vi "StateSpaceUtil_MakeCostMatrix.vi"(7 "Elements":i32, 11 "Costs":T1) -> (0 "Sze Coerced":bool, 3 "Costs Matrix":T1)   [LabVIEW 2019, in "Trajectory_Library.lvlib"]
doc: "Creates a cost matrix from the given vector for use with LQR.\n\nThe cost matrix is constructed using Bryson's rule. The inverse square of each tolerance is placed on the cost matrix diagonal. If a tolerance is infinity, its cost matrix entry is set to zero.\n \nInputs:\n - Elements -- representing the number of system states or inputs\n - tolerances -- For a Q matrix, its elements are the maximum allowed excursions of the states from the reference. For an R matrix, its elements are the maximum allowed excursions of the control inputs from no actuation.\n\nOutputs:\n - CostsMatrix -- State excursion or control effort cost matrix.\n - sizeCoerced -- If TRUE, an error occured."
uses:
  Trajectory_Library.lvlib
  <vilib>/Analysis/Matrix/Datatypes/RealMatrix.ctl
  <vilib>/Analysis/Matrix/NI_Matrix.lvlib
panel:
  # "<Elements,Elements>"
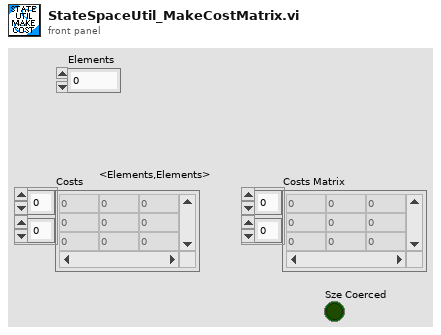
[diagram p1: front panel]
types:
  T1 = typedef "NI_Matrix.lvlib/RealMatrix.ctl" = dbl[][]
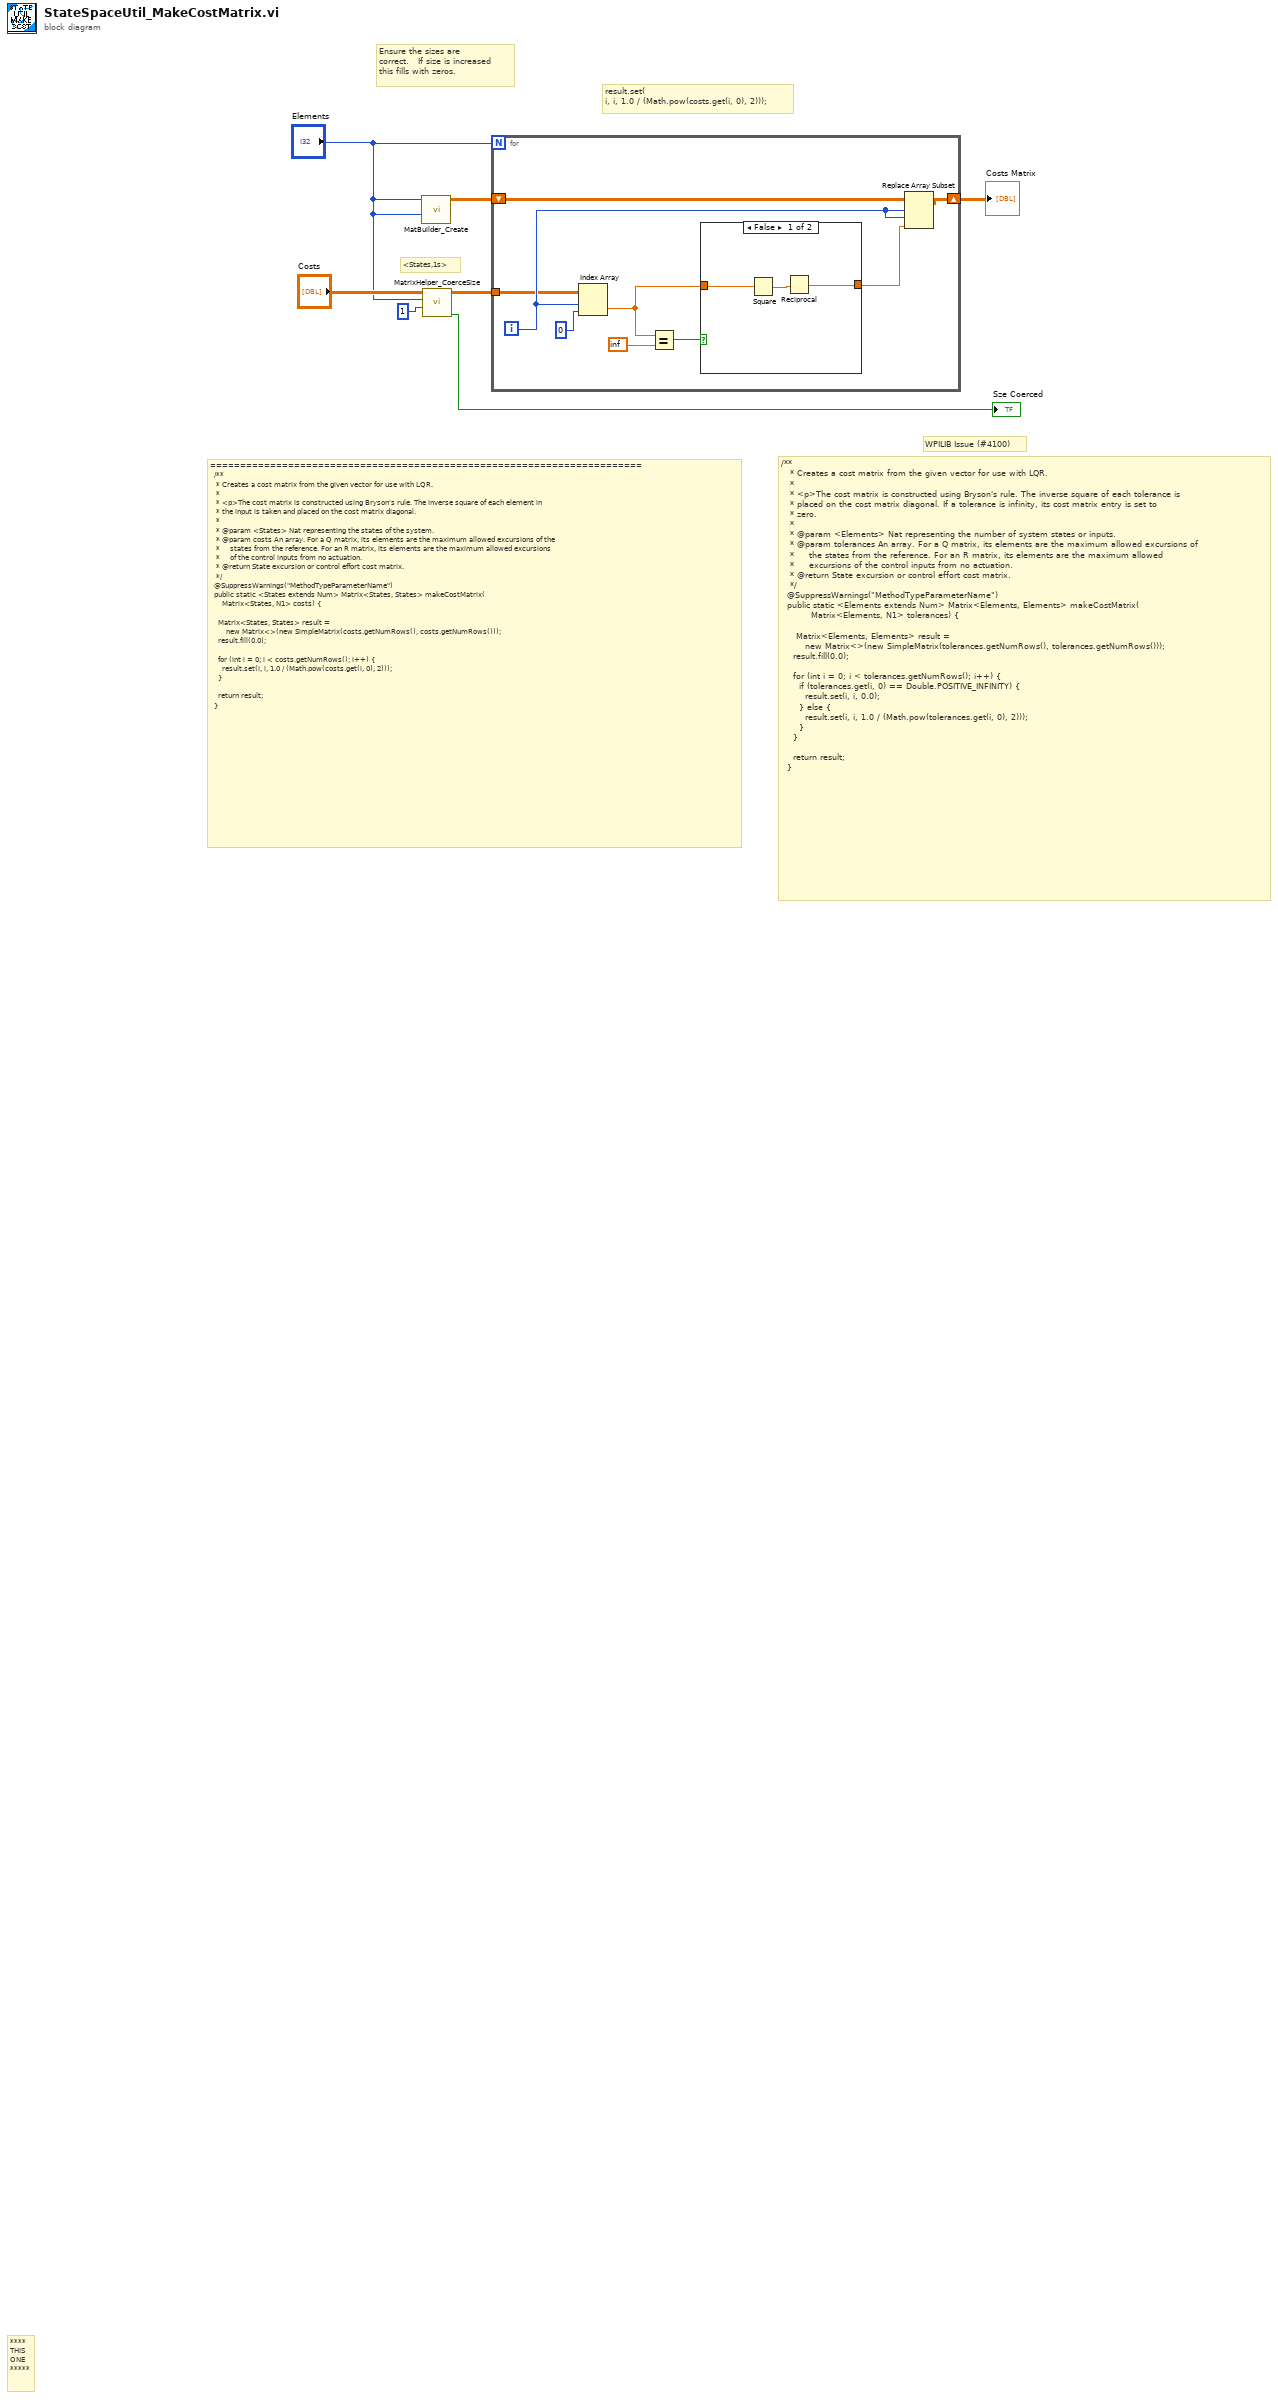
[diagram p0: block diagram]
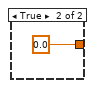
[diagram p2: hidden frame]
diagram:
  # "WPILIB Issue (#4100)"
  # "/**\n   * Creates a cost matrix from the given vector for use with LQR.\n   *\n   * <p>The cost matrix is constructed using Bryson's rule. The inverse square of each tolerance is\n   * placed on the cost matrix diagonal. If a tolerance is infinity, its cost matrix entry is set to\n   * zero.\n   *\n   * @param <Elements> Nat representing the number of system states or inputs.\n   * @param tolerances An array. For a Q matrix, its elements are the maximum allowed excursions of\n   *     the states from the reference. For an R matrix, its elements are the maximum allowed\n   *     excursions of the control inputs from no actuation.\n   * @return State excursion or control effort cost matrix.\n   */\n  @SuppressWarnings(\"MethodTypeParameterName\")\n  public static <Elements extends Num> Matrix<Elements, Elements> makeCostMatrix(\n      \t\t\t\tMatrix<Elements, N1> tolerances) {\n\n    \tMatrix<Elements, Elements> result =\n        new Matrix<>(new SimpleMatrix(tolerances.getNumRows(), tolerances.getNumRows()));\n    result.fill(0.0);\n\n    for (int i = 0; i < tolerances.getNumRows(); i++) {\n      if (tolerances.get(i, 0) == Double.POSITIVE_INFINITY) {\n        result.set(i, i, 0.0);\n      } else {\n        result.set(i, i, 1.0 / (Math.pow(tolerances.get(i, 0), 2)));\n      }\n    }\n\n    return result;\n  }"
  # "result.set(\ni, i, 1.0 / (Math.pow(costs.get(i, 0), 2)));"
  # "========================================================================\n  /**\n   * Creates a cost matrix from the given vector for use with LQR.\n   *\n   * <p>The cost matrix is constructed using Bryson's rule. The inverse square of each element in\n   * the input is taken and placed on the cost matrix diagonal.\n   *\n   * @param <States> Nat representing the states of the system.\n   * @param costs An array. For a Q matrix, its elements are the maximum allowed excursions of the\n   *     states from the reference. For an R matrix, its elements are the maximum allowed excursions\n   *     of the control inputs from no actuation.\n   * @return State excursion or control effort cost matrix.\n   */\n  @SuppressWarnings(\"MethodTypeParameterName\")\n  public static <States extends Num> Matrix<States, States> makeCostMatrix(\n      Matrix<States, N1> costs) {\n\n    Matrix<States, States> result =\n        new Matrix<>(new SimpleMatrix(costs.getNumRows(), costs.getNumRows()));\n    result.fill(0.0);\n\n    for (int i = 0; i < costs.getNumRows(); i++) {\n      result.set(i, i, 1.0 / (Math.pow(costs.get(i, 0), 2)));\n    }\n\n    return result;\n  }"
  # "<States,1s>"
  # "Ensure the sizes are\ncorrect.   If size is increased \nthis fills with zeros."
  # "****\nTHIS\nONE\n*****"
  n1 = call "MatBuilder_Create.vi"("Columns"="Elements", "Rows"="Elements") -> ("output matrix"=w3:T1)  [unwired: 9 in]
  n2 = call "MatrixHelper_CoerceSize.vi"("Columns"=1 ("number of columns"), "Rows"="Elements", "input matrix"="Costs") -> ("Coerced"=→"Sze Coerced":bool, "output matrix"=w2:T1)  [unwired: 7 in]
  n3 = for {
    N: "Elements" -> [_]
    tunnel: w2 -> [w12]
    shift-right: [w16] -> w7
    shift-left: w3 -> [w15]
    i -> [w14]
    n4 = Index Array(array=w12, index (row)=w14, index (col)=0) -> (element=w8:dbl)
    n5 = Equal?(x=w8, y=inf) -> (x = y?=w10:bool)
    n6 = case shown="False" w10 {
      tunnel: [w18 0.0] -> w9
      tunnel: w8 -> [w17 _]
      frame False {
        n7 = Square(x=w17) -> (x^2=w19:dbl)
        n8 = Reciprocal(x=w19) -> (1/x=w18:dbl)
      }
      frame True {
      }
    }
    n9 = Replace Array Subset(array=w15, new element=w9, index (row)=w14, index (col)=w14) -> (w16:T1)
  }
  "Costs Matrix" <- w7
